vi "VIH Dialog - VI Terminals - Coords to Control Index.vi"(10 "Coords":cluster{"Horizontal":i32, "Vertical":i32}, 11 "Controls info":T1(array[cluster])) -> (0 "Index":i32, 3 "dup Controls info":T1(array[cluster]))   [LabVIEW 2014]
doc: "::: VI Helpeks :::\nCopyright (c) 2000-2026 Konstantin Shifershteyn. All rights reserved."
panel:
  # "VI Helpeks\nCopyright (c) 2012-2026 Konstantin Shifershteyn"
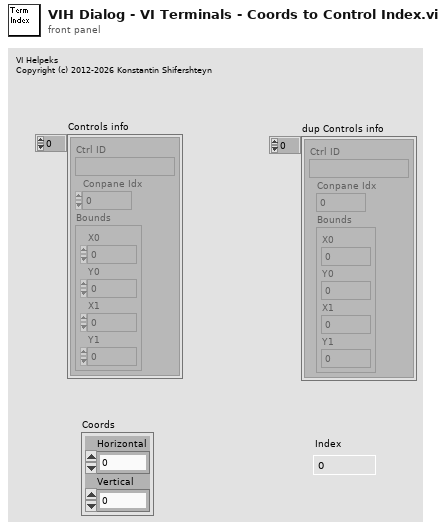
[diagram p1: front panel]
types:
  T1 = cluster{"Ctrl ID":string, "Conpane Idx":i32, "Bounds":cluster{"X0":i32, "Y0":i32, "X1":i32, "Y1":i32}}[]
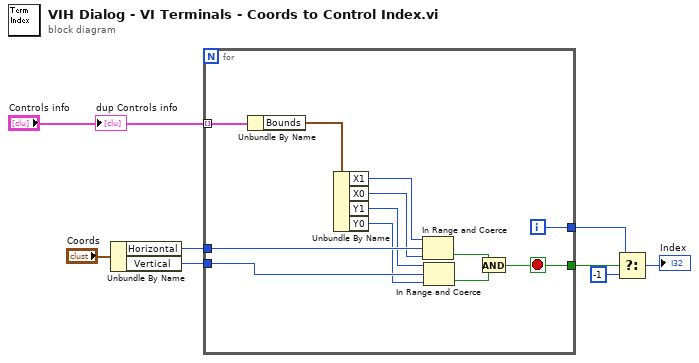
[diagram p0: block diagram]
diagram:
  n1 = Unbundle By Name("Coords") -> ("Horizontal"=w7:i32, "Vertical"=w6:i32)
  n2 = for {
    tunnel: "Controls info" -> [w20] mode=indexing
    tunnel: w7 -> [w18]
    tunnel: w6 -> [w17]
    tunnel: [w10] -> w5
    tunnel: [w9] -> w4
    i -> [w9]
    stop <- w10 stop-if-true
    n3 = Unbundle By Name(w20) -> ("Bounds"=w19:cluster{"X0":i32, "Y0":i32, "X1":i32, "Y1":i32})
    n4 = Unbundle By Name(w19) -> ("X1"=w16:i32, "X0"=w15:i32, "Y1"=w14:i32, "Y0"=w13:i32)
    n5 = In Range and Coerce(upper limit=w16, x=w18, lower limit=w15) -> (In Range?=w12:bool)  [unwired: 1 out]
    n6 = In Range and Coerce(upper limit=w14, x=w17, lower limit=w13) -> (In Range?=w11:bool)  [unwired: 1 out]
    n7 = And(x=w12, y=w11) -> (x .and. y?=w10:bool)
  }
  n8 = Select(t=w4, s=w5, f=-1) -> (s? t:f=→"Index":i32)
  "dup Controls info" <- "Controls info"
